vi "Handmatige besturing met druksensoruitlezing.vi"() -> ()   [LabVIEW 2024]
uses:
  <vilib>/DAQmx/write.llb/DAQmx Write (Digital 1D Bool NChan 1Samp 1Line).vi
  <vilib>/DAQmx/write.llb/DAQmx Write (Analog DBL 1Chan 1Samp).vi
  <vilib>/DAQmx/create/channels.llb/DAQmx Create Channel (AO-Voltage-Basic).vi
  <vilib>/DAQmx/miscellaneous.llb/DAQmx Fill In Error Info.vi
panel:
  in  "Boolean":bool
  out "Waveform Chart":dynamicdata(graph)
  in  "Analog output pressure regulator":tag="Dev1/ao0"
  in  "Set pressure Hybrid Heart (Bar)":dbl min=0.0 max=1.0 step=0.1
  in  "Seconds per data point":dbl
  out "data":dynamicdata(graph)
  in  "stop (F)":bool
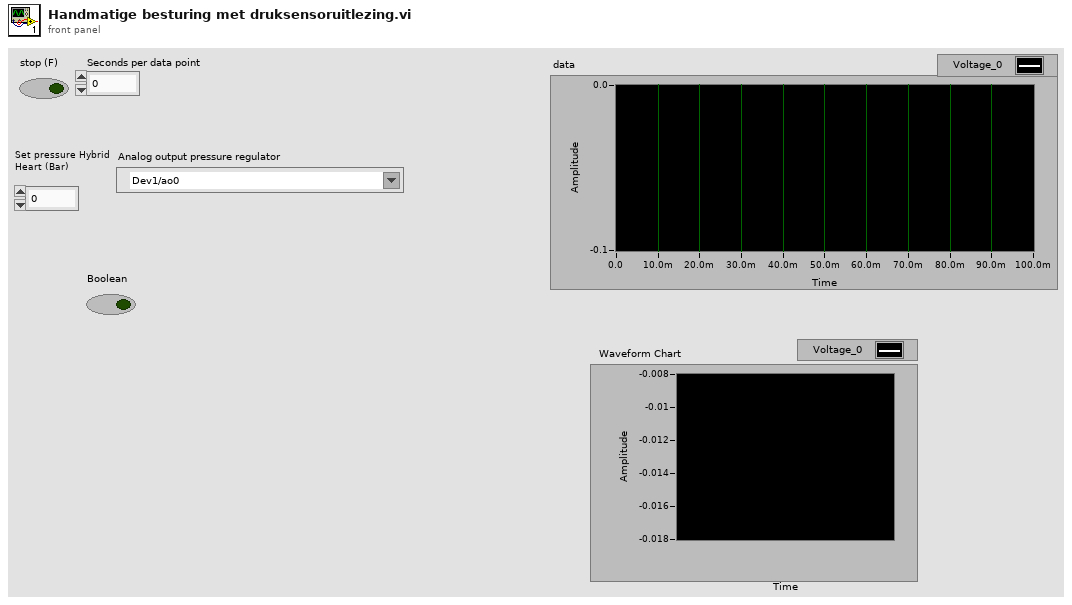
[diagram p1: front panel]
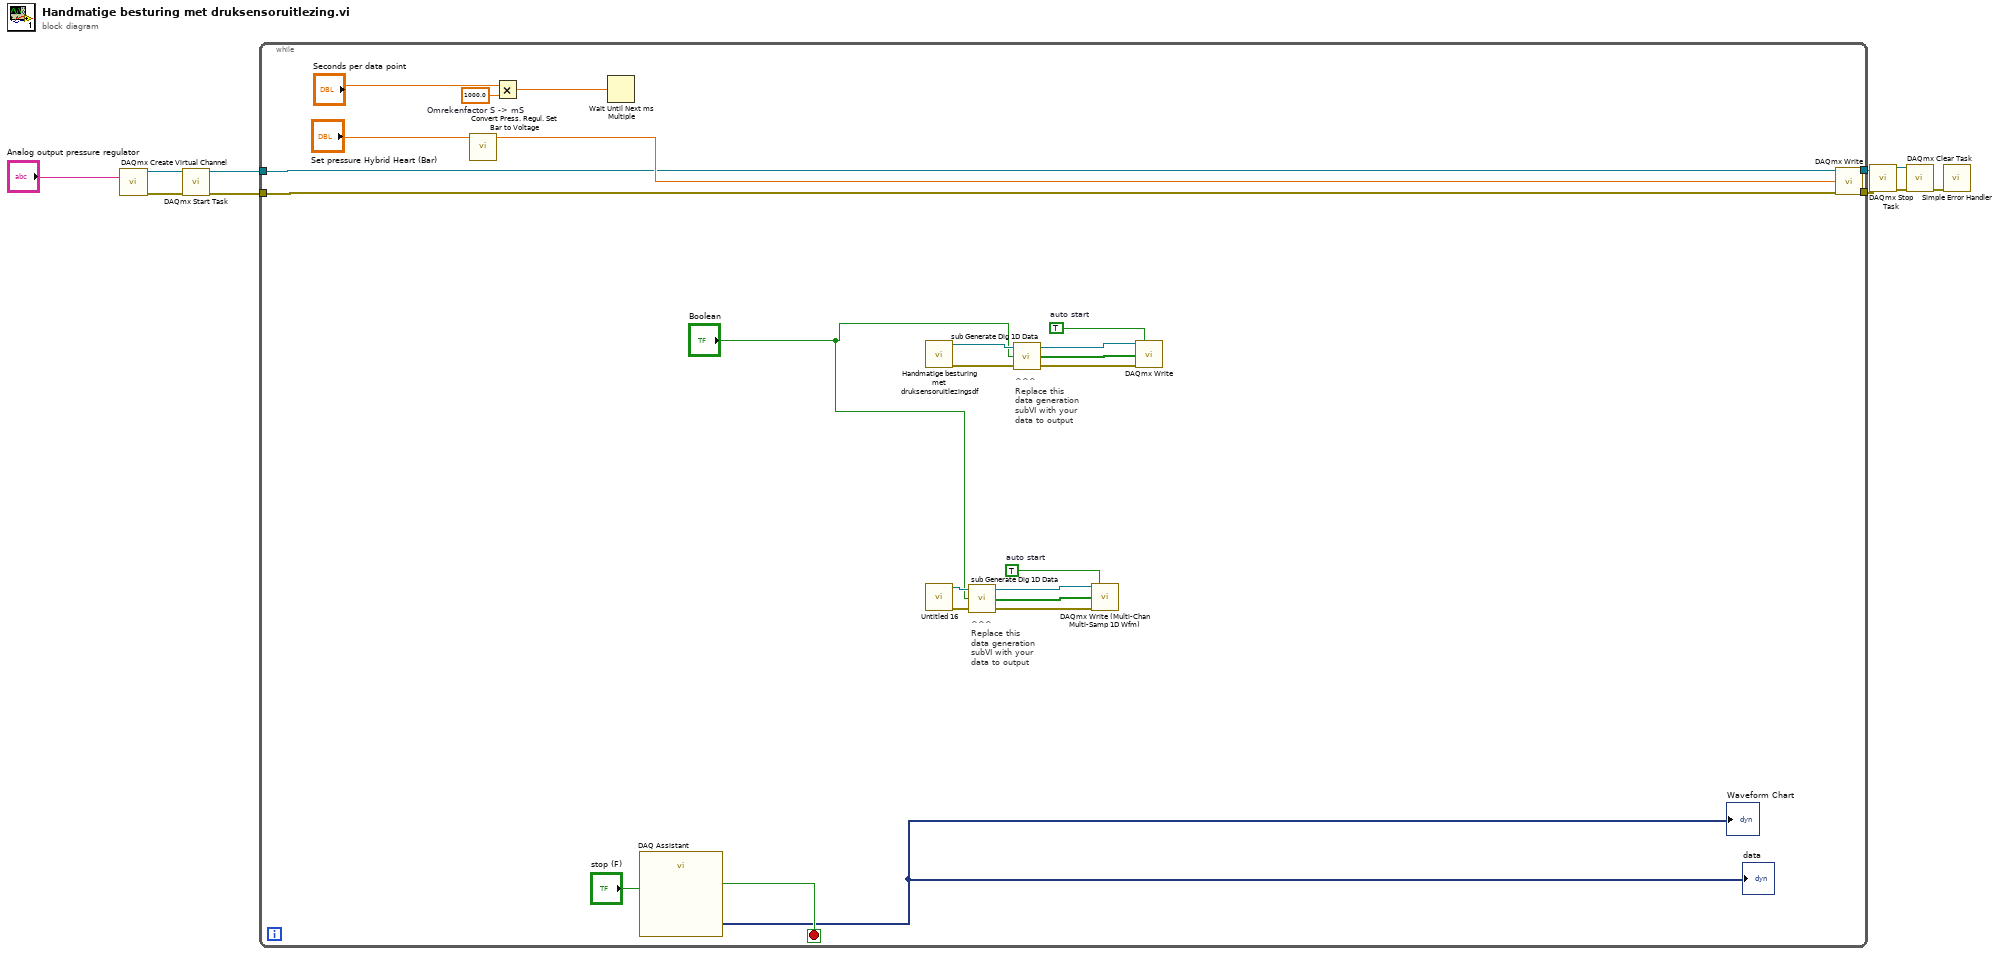
[diagram p0: block diagram]
diagram:
  n1 = call-poly <vilib>:"DAQmx Create Virtual Channel.vi"("physical channels"="Analog output pressure regulator") -> ("task out"=w7:refnum<k21>, "error out"=w6:errorcluster)  [unwired: 13 in]
  n2 = call <vilib>:"DAQmx Start Task.vi"("task/channels in"=w7, "error in"=w6) -> ("task out"=w3:refnum<k21>, "error out"=w4:errorcluster)  [unwired: 12 in]
  n3 = while {
    tunnel: w3 -> [w28]
    tunnel: w4 -> [w27]
    tunnel: [w26] -> w2
    tunnel: [w25] -> w1
    stop <- w34 stop-if-true
    w17 = TRUE  # auto start
    w23 = TRUE  # auto start
    w29 = 1000.0  # Omrekenfactor S -> mS
    # "^^^\nReplace this\ndata generation\nsubVI with your\ndata to output"
    # "^^^\nReplace this\ndata generation\nsubVI with your\ndata to output"
    n4 = call "Convert Press. Regul. Set Bar to Voltage.vi"("Set pressure Hybrid Heart (Bar)"="Set pressure Hybrid Heart (Bar)") -> ("Numeric"=w33:dbl)  [unwired: 10 in]
    n5 = Multiply(x="Seconds per data point", y=w29) -> (x*y=w30:dbl)
    n6 = Wait Until Next ms Multiple(millisecond multiple=w30) -> ()  [unwired: 1 out]
    n7 = call "DAQ Assistant"("stop (F)"="stop (F)") -> ("data"=→"data" →"Waveform Chart":dynamicdata, "stopped"=w34:bool)  [unwired: 15 in, 2 out]
    n8 = call "Handmatige besturing met druksensoruitlezingsdf.vi"() -> ("error out"=w18:errorcluster, "task out"=w19:refnum<k21>)  [unwired: 10 in]
    n9 = call "Untitled 16.vi"() -> ("error out"=w12:errorcluster, "task out"=w13:refnum<k21>)  [unwired: 10 in]
    n10 = call <vilib>:"sub Generate Dig 1D Data.vi"("error in"=w12, "initial value"="Boolean", "task in"=w13) -> ("error out"=w16:errorcluster, "Data"=w15:bool[], "task out"=w14:refnum<k21>)
    n11 = call <vilib>:"sub Generate Dig 1D Data.vi"("error in"=w18, "initial value"="Boolean", "task in"=w19) -> ("error out"=w22:errorcluster, "Data"=w21:bool[], "task out"=w20:refnum<k21>)
    n12 = call-poly "DAQmx Write (Multi-Chan Multi-Samp 1D Wfm).vi"("task/channels in"=w14, "auto start"=w17, "data"=w15, "error in"=w16) -> ()  [unwired: 9 in, 3 out]
    n13 = call-poly <vilib>:"DAQmx Write.vi"("task/channels in"=w20, "auto start"=w23, "data"=w21, "error in"=w22) -> ()  [unwired: 9 in, 3 out]
    n14 = call-poly <vilib>:"DAQmx Write.vi"("task/channels in"=w28, "data"=w33, "error in"=w27) -> ("task out"=w25:refnum<k21>, "error out"=w26:errorcluster)  [unwired: 10 in, 1 out]
  }
  n15 = call <vilib>:"DAQmx Stop Task.vi"("task/channels in"=w1, "error in"=w2) -> ("task out"=w9:refnum<k21>, "error out"=w10:errorcluster)  [unwired: 12 in]
  n16 = call <vilib>:"DAQmx Clear Task.vi"("task in"=w9, "error in"=w10) -> ("error out"=w8:errorcluster)  [unwired: 13 in]
  n17 = call <vilib>:"Simple Error Handler.vi"("error in (no error)"=w8) -> ()  [unwired: 4 in, 5 out]
